vi "connectNodes.vi"(0 "reference":refnum<class "Graph.lvclass">, 1 "egde":refnum<class "AbstractEdge.lvclass">, 2 "start":refnum<class "AbstractNode.lvclass">, 3 "end":refnum<class "AbstractNode.lvclass">, 5 "error in (no error)":errorcluster) -> (14 "reference out":refnum<class "Graph.lvclass">, 15 "connected":bool, 19 "error out":errorcluster)   [LabVIEW 2020, in "Graph.lvclass"]
uses:
  <resource>/Framework/Providers/Open_GDS/UML/Graph_class/Graph.lvclass
  <resource>/Framework/Providers/Open_GDS/UML/AbstractEdge_class/AbstractEdge.lvclass
  <resource>/Framework/Providers/Open_GDS/UML/AbstractNode_class/AbstractNode.lvclass
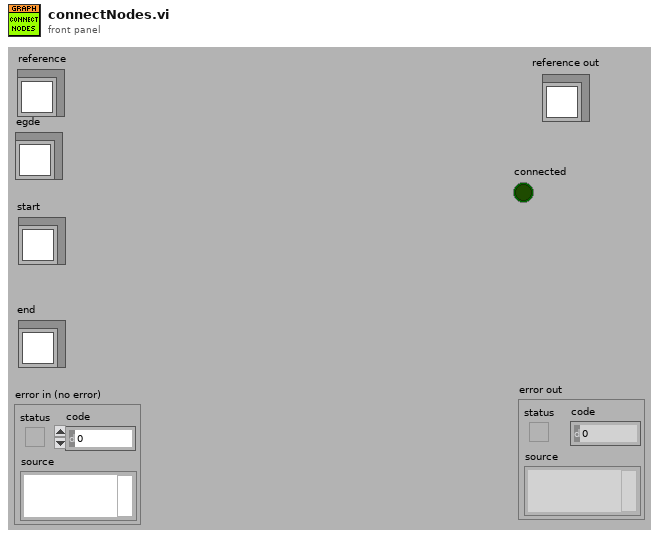
[diagram p1: front panel]
types:
  T1 = typedef "Graph.lvclass/ObjectAttributes.ctl" = cluster{"nodes":refnum<class "AbstractNode.lvclass">[], "edges":refnum<class "AbstractEdge.lvclass">[], "nodesToBeRemoved":refnum<class "AbstractNode.lvclass">[], "edgesToBeRemoved":refnum<class "AbstractEdge.lvclass">[], "needsLayout":bool, "LayoutNodes":refnum<class "AbstractNode.lvclass">[]}
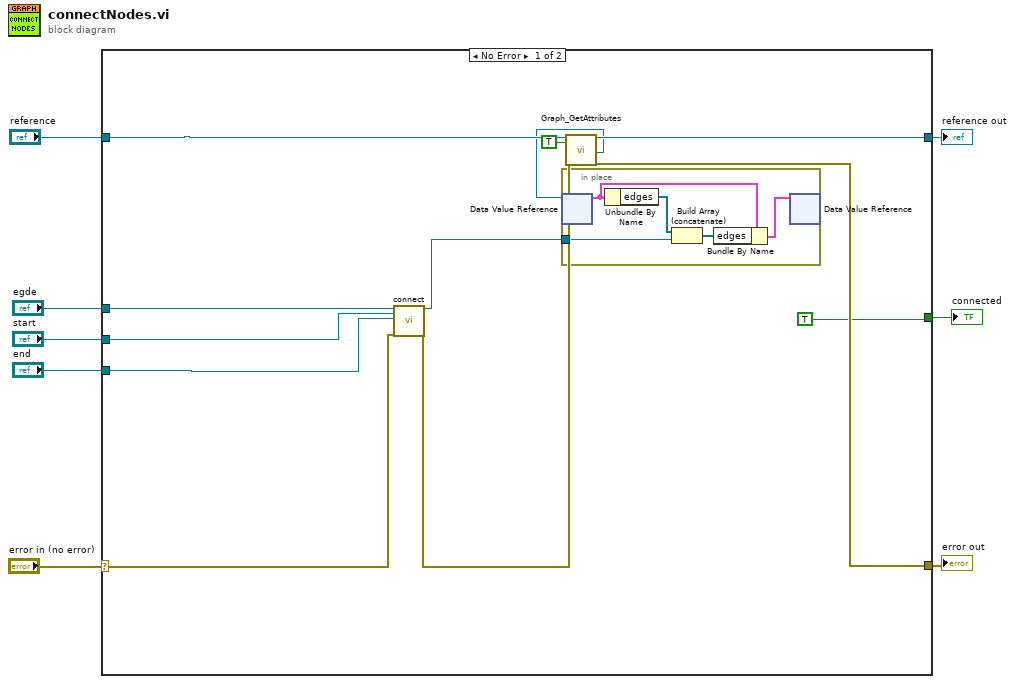
[diagram p0: block diagram]
diagram:
  n1 = case shown="No Error" "error in (no error)" {
    selector: "error in (no error)" -> [w17 w26]
    tunnel: "reference" -> [w20 w27]
    tunnel: [w19 w26] -> w7
    tunnel: [w18 w27] -> w6
    tunnel: "egde" -> [w16 _]
    tunnel: "start" -> [w15 _]
    tunnel: "end" -> [w14 _]
    tunnel: [TRUE ("needsLayout") _] -> w1
    frame No Error {
      n2 = call-dynamic "connect.vi"("reference"=w16, "startNode"=w15, "endNode"=w14, "error in (no error)"=w17) -> ("reference out"=w9:refnum<class "AbstractEdge.lvclass">, "error out"=w12:errorcluster)  [unwired: 14 out]
      n3 = call <resource>:"Graph_GetAttributes.vi"("reference in"=w20, "OnlyGetDvrReference(False)"=TRUE, "error in (no error)"=w12) -> ("reference out"=w18:refnum<class "Graph.lvclass">, "DataRef"=w10:refnum<data-value>, "error out"=w19:errorcluster)  [unwired: 13 in, 1 out]
      n4 = in-place {
        in-place-border: w9 -> [w21]
        n5 = in-place-dvr #1(w10) -> (w25:T1)  [unwired: 1 out]
        n6 = Unbundle By Name(w25) -> ("edges"=w24:refnum<class "AbstractEdge.lvclass">[])
        n7 = Build Array (concatenate)(w24, w21) -> (w23:refnum<class "AbstractEdge.lvclass">[])
        n8 = Bundle By Name(cluster=w25, "edges"=w23) -> (w22:T1)
        n9 = in-place-dvr #1(w22) -> ()  [unwired: 2 out]
      }
    }
    frame Error {
    }
  }
  "reference out" <- w6
  "error out" <- w7
  "connected" <- w1
